vi "test prompt required argument.vi"(8 "error in (no error)":errorcluster) -> (0 "error out":errorcluster, 3 "body":string)   [LabVIEW 2020, in "MCP Server tests.lvlib"]
doc: "prompts/get without a required argument is answered with JSON-RPC error -32602 that names the argument. With the argument the prompt is returned and contains the value."
uses:
  MCP Server tests.lvlib
  <vilib>/JDP Science/JSONtext/Next JSON Value.vi
  <vilib>/JDP Science/JSONtext/String Subset.vi
  <vilib>/JDP Science/JSONtext/Parsing/Advance past next JSON Value (inlined COPY).vi
  <vilib>/JDP Science/JSONtext/Parsing/Advance past whitespace.vi
  <vilib>/JDP Science/JSONtext/Parsing/Advance past String.vi
  <vilib>/JDP Science/JSONtext/Parsing/Advance past Number.vi
  <vilib>/JDP Science/JSONtext/Parsing/Advance past Line Ending.vi
  <vilib>/JDP Science/JSONtext/Parsing/Parse Full Path or Item Name.vi
  <vilib>/JDP Science/JSONtext/Parsing/Advance past Array.vi
  <vilib>/JDP Science/JSONtext/Parsing/Advance past Object.vi
  <vilib>/JDP Science/JSONtext/support/Error Cluster From Code.vi
  <vilib>/JDP Science/JSONtext/Offset/Find Item Locations by Path.vi
  <vilib>/addons/_JKI Toolkits/Caraya/classes/Test/Test.lvclass
  <vilib>/JDP Science/JSONtext/JSONtext.lvlib
  <vilib>/addons/_JKI Toolkits/Caraya/classes/Assert/Assert.lvclass
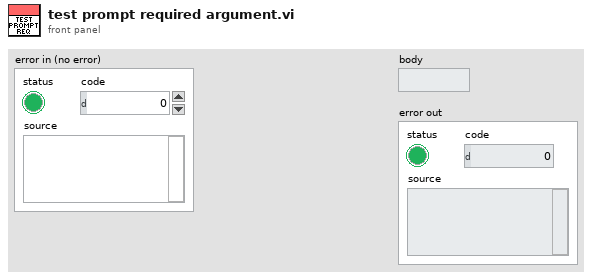
[diagram p1: front panel]
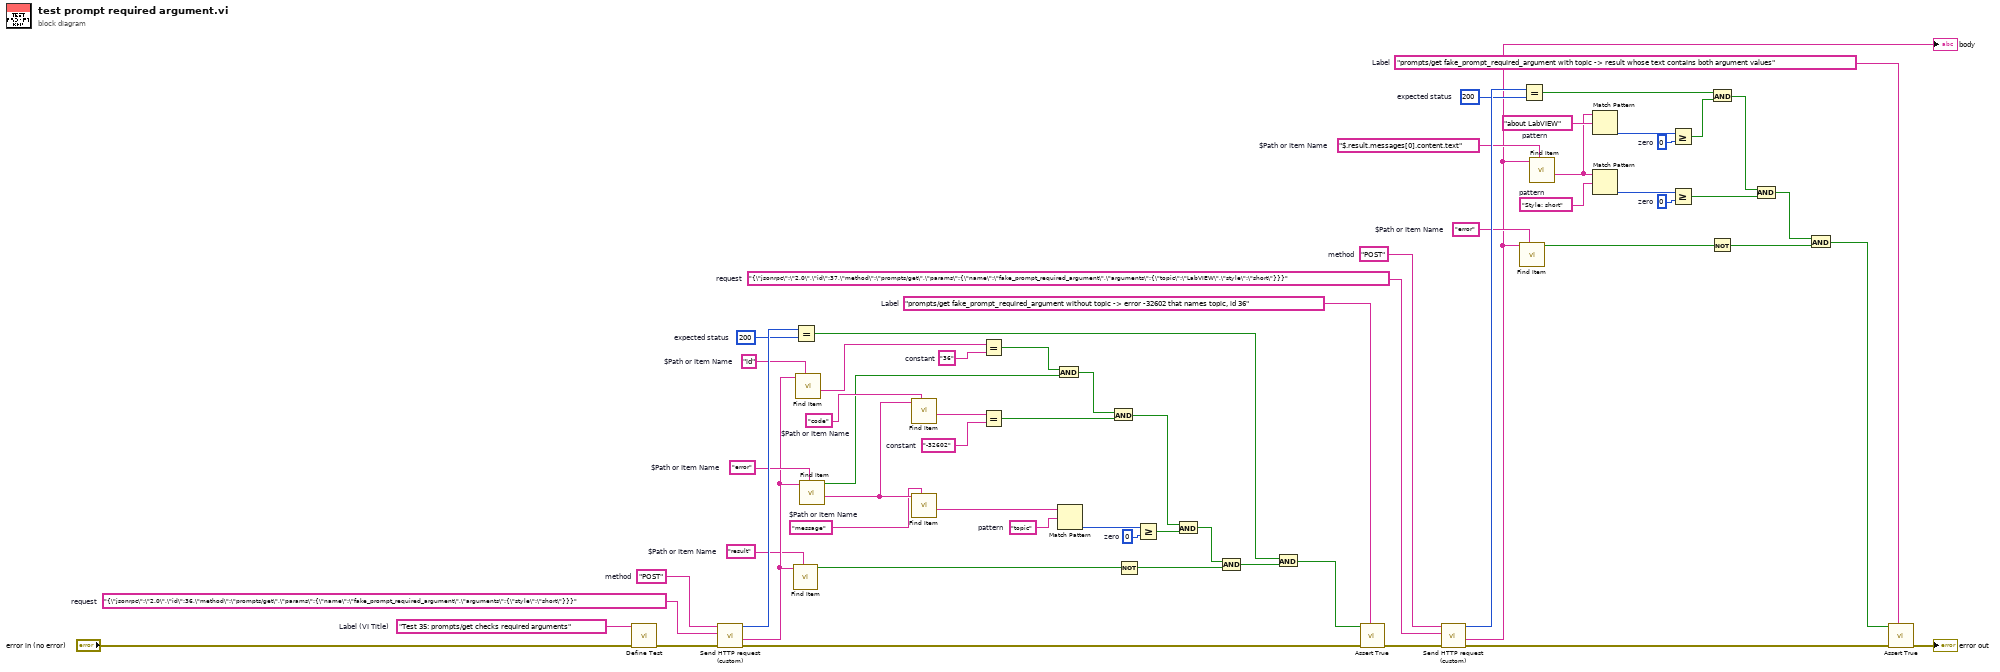
[diagram p0: block diagram]
diagram:
  w3 = "prompts/get fake_prompt_required_argument with topic -> result whose text contains both argument values"  # Label
  w13 = 0  # zero
  w15 = "Style: short"  # pattern
  w17 = 0  # zero
  w19 = "about LabVIEW"  # pattern
  w20 = "error"  # $Path or Item Name
  w21 = "$.result.messages[0].content.text"  # $Path or Item Name
  w22 = 200  # expected status
  w25 = "{\"jsonrpc\":\"2.0\",\"id\":37,\"method\":\"prompts/get\",\"params\":{\"name\":\"fake_prompt_required_argument\",\"arguments\":{\"topic\":\"LabVIEW\",\"style\":\"short\"}}}"  # request
  w26 = "POST"  # method
  w27 = "prompts/get fake_prompt_required_argument without topic -> error -32602 that names topic, id 36"  # Label
  w41 = 0  # zero
  w43 = "topic"  # pattern
  w45 = "-32602"  # constant
  w47 = "36"  # constant
  w49 = "result"  # $Path or Item Name
  w51 = "message"  # $Path or Item Name
  w53 = "code"  # $Path or Item Name
  w54 = "error"  # $Path or Item Name
  w55 = "id"  # $Path or Item Name
  w56 = 200  # expected status
  w59 = "{\"jsonrpc\":\"2.0\",\"id\":36,\"method\":\"prompts/get\",\"params\":{\"name\":\"fake_prompt_required_argument\",\"arguments\":{\"style\":\"short\"}}}"  # request
  w60 = "POST"  # method
  w62 = "Test 35: prompts/get checks required arguments"  # Label (VI Title)
  n1 = call <vilib>:"Define Test.vi"("error in (no error)"="error in (no error)", "Label (VI Title)"=w62) -> ("error out"=w58:errorcluster)  [unwired: 8 in, 1 out]
  n2 = call "Send HTTP request (custom).vi"("error in (no error)"=w58, "request"=w59, "method"=w60) -> ("error out"=w28:errorcluster, "response"=w50:string, "status code"=w57:i32)  [unwired: 5 in, 1 out]
  n3 = call <vilib>:"Find Item.vi"("$Path or Item Name"=w49, "JSON"=w50) -> ("Found"=w40:bool)  [unwired: 6 in, 3 out]
  n4 = Equal?(x=w57, y=w56) -> (x = y?=w31:bool)
  n5 = call <vilib>:"Find Item.vi"("$Path or Item Name"=w55, "JSON"=w50) -> ("<JSON>"=w48:string)  [unwired: 6 in, 3 out]
  n6 = call <vilib>:"Find Item.vi"("$Path or Item Name"=w54, "JSON"=w50) -> ("<JSON>"=w52:string, "Found"=w38:bool)  [unwired: 6 in, 2 out]
  n7 = call <vilib>:"Find Item.vi"("$Path or Item Name"=w53, "JSON"=w52) -> ("<JSON>"=w46:string)  [unwired: 6 in, 3 out]
  n8 = call <vilib>:"Find Item.vi"("$Path or Item Name"=w51, "JSON"=w52) -> ("<JSON>"=w44:string)  [unwired: 6 in, 3 out]
  n9 = Equal?(x=w48, y=w47) -> (x = y?=w39:bool)
  n10 = Equal?(x=w46, y=w45) -> (x = y?=w36:bool)
  n11 = And(x=w39, y=w38) -> (x .and. y?=w37:bool)
  n12 = Match Pattern(string=w44, regular expression=w43) -> (offset past match=w42:i32)  [unwired: 1 in, 3 out]
  n13 = And(x=w37, y=w36) -> (x .and. y?=w35:bool)
  n14 = Not(x=w40) -> (.not. x?=w32:bool)
  n15 = Greater Or Equal?(x=w42, y=w41) -> (x >= y?=w34:bool)
  n16 = And(x=w35, y=w34) -> (x .and. y?=w33:bool)
  n17 = And(x=w33, y=w32) -> (x .and. y?=w30:bool)
  n18 = And(x=w31, y=w30) -> (x .and. y?=w29:bool)
  n19 = call <vilib>:"Assert True.vi"("Label"=w27, "error in (no error)"=w28, "True?"=w29) -> ("error out"=w24:errorcluster)  [unwired: 7 in, 1 out]
  n20 = call "Send HTTP request (custom).vi"("error in (no error)"=w24, "request"=w25, "method"=w26) -> ("error out"=w4:errorcluster, "response"=w2:string, "status code"=w23:i32)  [unwired: 5 in, 1 out]
  "body" <- w2
  n21 = call <vilib>:"Find Item.vi"("$Path or Item Name"=w20, "JSON"=w2) -> ("Found"=w12:bool)  [unwired: 6 in, 3 out]
  n22 = Equal?(x=w23, y=w22) -> (x = y?=w11:bool)
  n23 = call <vilib>:"Find Item.vi"("$Path or Item Name"=w21, "JSON"=w2) -> ("<JSON>"=w16:string)  [unwired: 6 in, 3 out]
  n24 = Match Pattern(string=w16, regular expression=w19) -> (offset past match=w18:i32)  [unwired: 1 in, 3 out]
  n25 = Match Pattern(string=w16, regular expression=w15) -> (offset past match=w14:i32)  [unwired: 1 in, 3 out]
  n26 = Greater Or Equal?(x=w18, y=w17) -> (x >= y?=w10:bool)
  n27 = Greater Or Equal?(x=w14, y=w13) -> (x >= y?=w8:bool)
  n28 = And(x=w11, y=w10) -> (x .and. y?=w9:bool)
  n29 = Not(x=w12) -> (.not. x?=w6:bool)
  n30 = And(x=w9, y=w8) -> (x .and. y?=w7:bool)
  n31 = And(x=w7, y=w6) -> (x .and. y?=w5:bool)
  n32 = call <vilib>:"Assert True.vi"("Label"=w3, "error in (no error)"=w4, "True?"=w5) -> ("error out"=→"error out":errorcluster)  [unwired: 7 in, 1 out]
